vi "Savitsky Golay Filter (multiple).vi"(6 "Side Points Unit (points)":enum16{"Points", "Data"}(ring), 8 "error in (no error)":errorcluster, 9 "polynomial order (3)":i32=3, 10 "side points (6)":dbl=6.0, 11 "XY-data":cluster{"X-array":dbl[], "Y-array":dbl[]}[](array[cluster])) -> (0 "error out":errorcluster, 3 "XY-data out":cluster{"X-array":dbl[], "Y-array":dbl[]}[](array[cluster]) {"Y-array" format="%.2p"; "X-array" format="%.2p"})   [LabVIEW 2019, in "xy_utilities.lvlib"]
doc: "Filter <b>XY-data</b>'s Y-Array with a Savitsky-Golay FIR smoothing filter.\n\n<b>side points</b> specifies the number of data points to each side of the current data point to use for the least squares minimization. side points*2 + 1 is the length of the moving window, which must be greater than the polynomial order.\n\n<b>polynomial order</b> specifies the order of the polynomial. \n\nWire data to the data input to determine the polymorphic instance to use or manually select the instance."
uses:
  xy_utilities.lvlib
  Private/X Units.vi
  <vilib>/Analysis/3filter.llb/Savitzky-Golay Filter.vi
  <vilib>/Analysis/3filter.llb/Savitzky-Golay Filter (DBL).vi
  Private/X Array Range to Index.vi
  <vilib>/Utility/error.llb/Error Cluster From Error Code.vi
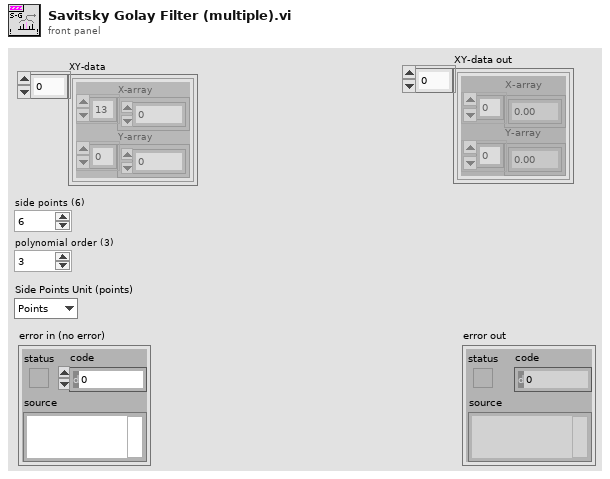
[diagram p1: front panel]
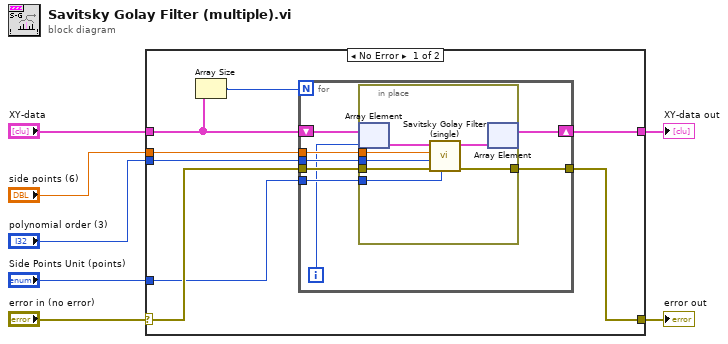
[diagram p0: block diagram]
diagram:
  n1 = case shown="No Error" "error in (no error)" {
    selector: "error in (no error)" -> [w13 w32]
    tunnel: [w12 w32] -> w6
    tunnel: "XY-data" -> [w8 w31]
    tunnel: [w15 w31] -> w4
    tunnel: "side points (6)" -> [w14 _]
    tunnel: "Side Points Unit (points)" -> [w11 _]
    tunnel: "polynomial order (3)" -> [w10 _]
    frame No Error {
      n2 = Array Size(array=w8) -> (size(s)=w9:i32)
      n3 = for {
        N: w9 -> [_]
        tunnel: w14 -> [w23]
        tunnel: w13 -> [w22]
        tunnel: [w21] -> w12
        tunnel: w11 -> [w20]
        tunnel: w10 -> [w19]
        shift-right: [w17] -> w15
        shift-left: w8 -> [w18]
        i -> [w16]
        n4 = in-place {
          in-place-border: w23 -> [w30]
          in-place-border: w22 -> [w29]
          in-place-border: [w28] -> w21
          in-place-border: w20 -> [w27]
          in-place-border: w19 -> [w26]
          n5 = in-place-array #1(w18, w16) -> (w25:cluster{"X-array":dbl[], "Y-array":dbl[]})
          n6 = call "Savitsky Golay Filter (single).vi"("Side Points Unit (points)"=w27, "error in (no error)"=w29, "polynomial order (3)"=w26, "side points (6)"=w30, "XY-data"=w25) -> ("error out"=w28:errorcluster, "XY-data out"=w24:cluster{"X-array":dbl[], "Y-array":dbl[]})  [unwired: 5 in]
          n7 = in-place-array #1(w24) -> (w17:cluster{"X-array":dbl[], "Y-array":dbl[]}[])  [unwired: 1 out]
        }
      }
    }
    frame Error {
    }
  }
  "error out" <- w6
  "XY-data out" <- w4
